vi "isInheritance.vi"(0 "reference":refnum<class "AbstractEdge.lvclass">, 5 "error in (no error)":errorcluster) -> (14 "reference out":refnum<class "AbstractEdge.lvclass">, 15 "isInheritance":bool, 16 "isCompAggregation":bool, 18 "isInterfaecImplementing":bool, 19 "error out":errorcluster)   [LabVIEW 2020, in "AbstractEdge.lvclass"]
doc: "Returns TRUE if Edge is a inheritance type"
uses:
  <resource>/Framework/Providers/Open_GDS/UML/AbstractEdge_class/AbstractEdge.lvclass
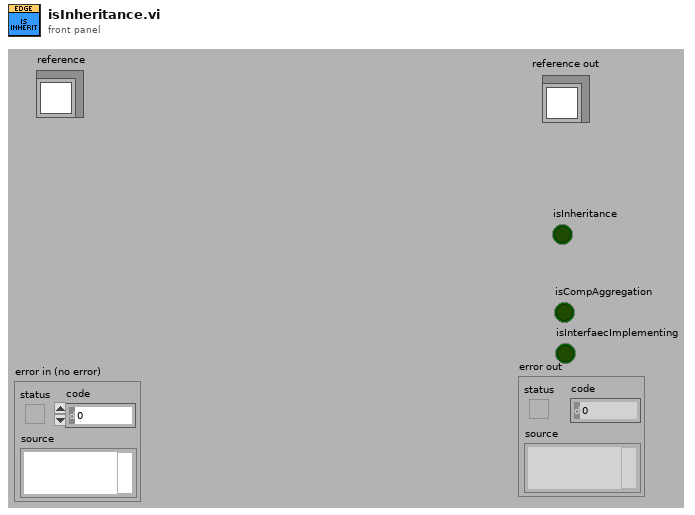
[diagram p1: front panel]
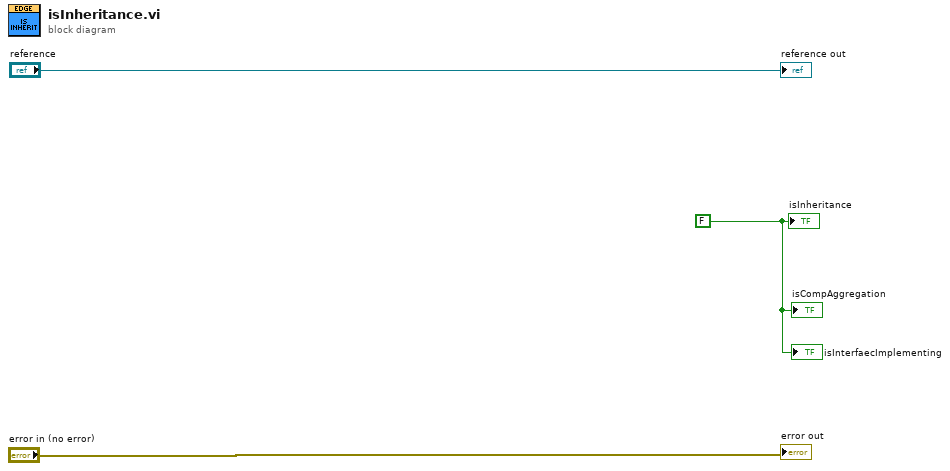
[diagram p0: block diagram]
diagram:
  w1 = FALSE ("isInheritance")
  "reference out" <- "reference"
  "error out" <- "error in (no error)"
  "isInheritance" <- w1
  "isCompAggregation" <- w1
  "isInterfaecImplementing" <- w1
